vi "Launch Connection Handler.vi"(8 "error in (no error)":errorcluster, 11 "Server in":refnum<class "Server.lvclass">) -> (0 "error out":errorcluster, 3 "Server out":refnum<class "Server.lvclass">)   [LabVIEW 2013, in "MQTT Server.lvlib" / "Server.lvclass"]
uses:
  Server.lvclass
  <vilib>/LabVIEW Open Source Project/MQTT Connection/MQTT_Base/Base Class/MQTT_Base.lvclass/MQTT_Base.ctl
  Server.lvclass/Server.ctl
  ConnectionHandler/ConnectionHandler.lvclass/ConnectionHandler.ctl
  <vilib>/LabVIEW Open Source Project/Connection/Connection/Connection.lvclass
  <vilib>/LabVIEW Open Source Project/MQTT Control Packets/Control Packets/ControlPacket/ControlPacket.lvclass
  ConnectionHandler/ConnectionHandler.lvclass
  <vilib>/LabVIEW Open Source Project/MQTT Connection/MQTT_Base/Base Class/MQTT_Base.lvclass
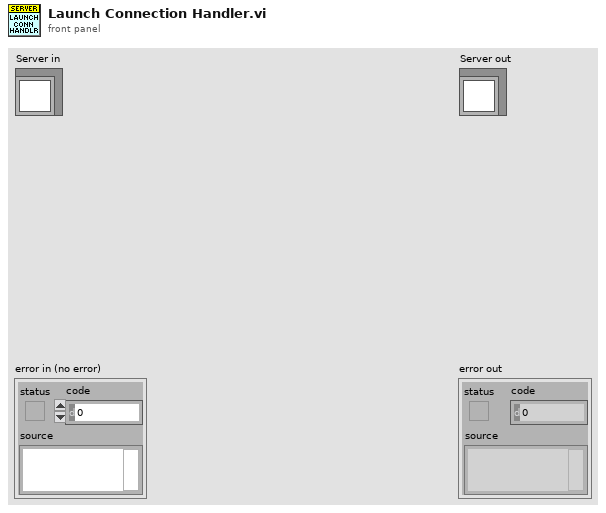
[diagram p1: front panel]
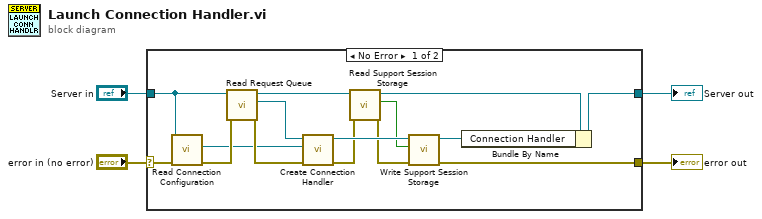
[diagram p0: block diagram]
diagram:
  n1 = case shown="No Error" "error in (no error)" {
    selector: "error in (no error)" -> [w15 w21]
    tunnel: [w8 w21] -> w3
    tunnel: [w19 w20] -> w1
    tunnel: "Server in" -> [w16 w20]
    frame No Error {
      n2 = call <vilib>:"Read Connection Configuration.vi"("error in (no error)"=w15, "MQTT_Base in"=w16) -> ("error out"=w14:errorcluster, "Connection Configuration"=w13:refnum<class "Connection.lvclass">)  [unwired: 7 in, 1 out]
      n3 = call <vilib>:"Read Request Queue.vi"("error in (no error)"=w14, "MQTT_Base in"=w16) -> ("error out"=w17:errorcluster, "Request"=w18:refnum<queue>, "MQTT_Base out"=w12:refnum<class "Server.lvclass">)  [unwired: 7 in]
      n4 = call "Create Connection Handler.vi"("error in (no error)"=w17, "Connection Configuration"=w13, "Request"=w18) -> ("error out"=w6:errorcluster, "ConnectionHandler"=w10:refnum<class "ConnectionHandler.lvclass">)  [unwired: 7 in]
      n5 = call "Read Support Session Storage.vi"("error in (no error)"=w6, "Server in"=w12) -> ("error out"=w5:errorcluster, "Support Session Storage"=w7:bool, "Server out"=w11:refnum<class "Server.lvclass">)  [unwired: 7 in]
      n6 = call "Write Support Session Storage.vi"("error in (no error)"=w5, "Support Session Storage"=w7, "ConnectionHandler in"=w10) -> ("error out"=w8:errorcluster, "ConnectionHandler out"=w9:refnum<class "ConnectionHandler.lvclass">)  [unwired: 7 in]
      n7 = Bundle By Name(cluster=w11, "Connection Handler"=w9) -> (w19:refnum<class "Server.lvclass">)
    }
    frame Error {
    }
  }
  "error out" <- w3
  "Server out" <- w1
